vi "XNET CAN2 Receive Probe.vi"(0 "interface":string="CAN2", 5 "database":string="eDyno_NVH_PoC", 7 "signals":string[](array[string])=["DYNO_Status.DynoSts_BlockCounter", "DYNO_Status.DynoSts_SpeedAct", "DYNO_Cmd.DynoCmd_Mode", "SIM_FaultStatus.FltSts_Freq_1x", "SIM_Config.SimCfg_SampleRate"]) -> (4 "values":dbl[](array[numeric]), 15 "error out":errorcluster)   [LabVIEW 2026]
doc: "Opens a Signal Input Single-point session on CAN2 with the eDyno_NVH_PoC alias (bus settings from the database), reads 20 times over ~2 s and returns the last values."
uses:
  <vilib>/xnet/xnet.llb/XNET Create Session (Generic).vi
  <vilib>/xnet/xnet.llb/XNET Read (Signal Single-point).vi
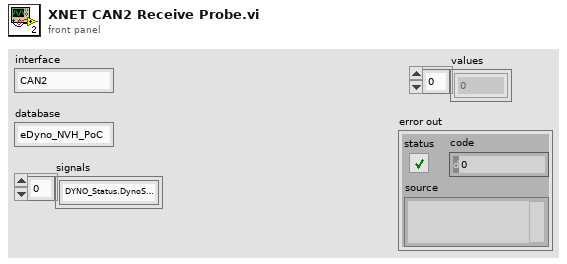
[diagram p1: front panel]
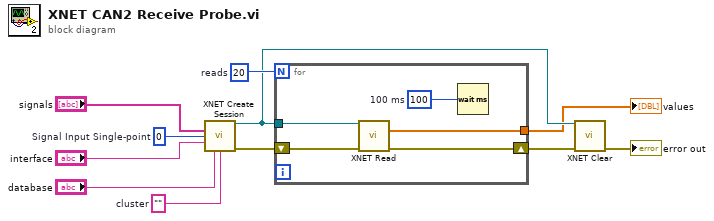
[diagram p0: block diagram]
diagram:
  w5 = 20  # reads
  w7 = ""  # cluster
  w10 = u32 0  # Signal Input Single-point
  n1 = call-poly <vilib>:"XNET Create Session.vi"("list (empty)"="signals", "mode"=w10, "interface"="interface", "database (:memory:)"="database", "cluster (empty)"=w7) -> ("session out"=w4:refnum<k21>, "error out"=w6:errorcluster)  [unwired: 9 in]
  n2 = for {
    N: w5 -> [_]
    tunnel: w4 -> [w15]
    tunnel: [w14] -> w2
    shift-right: [w13] -> w3
    shift-left: w6 -> [w12]
    w16 = 100  # 100 ms
    n3 = call-poly <vilib>:"XNET Read.vi"("session in"=w15, "error in (no error)"=w12) -> ("data"=w14:dbl[], "error out"=w13:errorcluster)  [unwired: 11 in, 1 out]
    n4 = Wait (ms)(milliseconds to wait=w16) -> ()  [unwired: 1 out]
  }
  "values" <- w2
  n5 = call <vilib>:"XNET Clear.vi"("session in"=w4, "error in (no error)"=w3) -> ("error out"=→"error out":errorcluster)  [unwired: 13 in]
